vi "N-216 Stage Engine.vi"(0 "Unique Notifier Name":string, 11 "COM Port":string[](array[string])) -> ()   [LabVIEW 2016]
uses:
  Stages Controls/Stage Focus Control.ctl
  Stages Controls/Stage Status.ctl
  Stages Controls/Stage Actions.ctl
  Stages Controls/Stage Notifier Element.ctl
  PI GCS2 DLL/PI_GCS2_DLL_x64.dll
panel:
  in  "Reference":bool
  in  "Velocity (µm/s)":dbl=0.1 format="%#_13g"
  out "Number Connected":i32
  out "E-712 Found":bool
  in  "ReInitialize":bool
  in  "Abort":bool
  out "Status":T1
  in  "QUIT":bool
  in  "Focus Control":T2
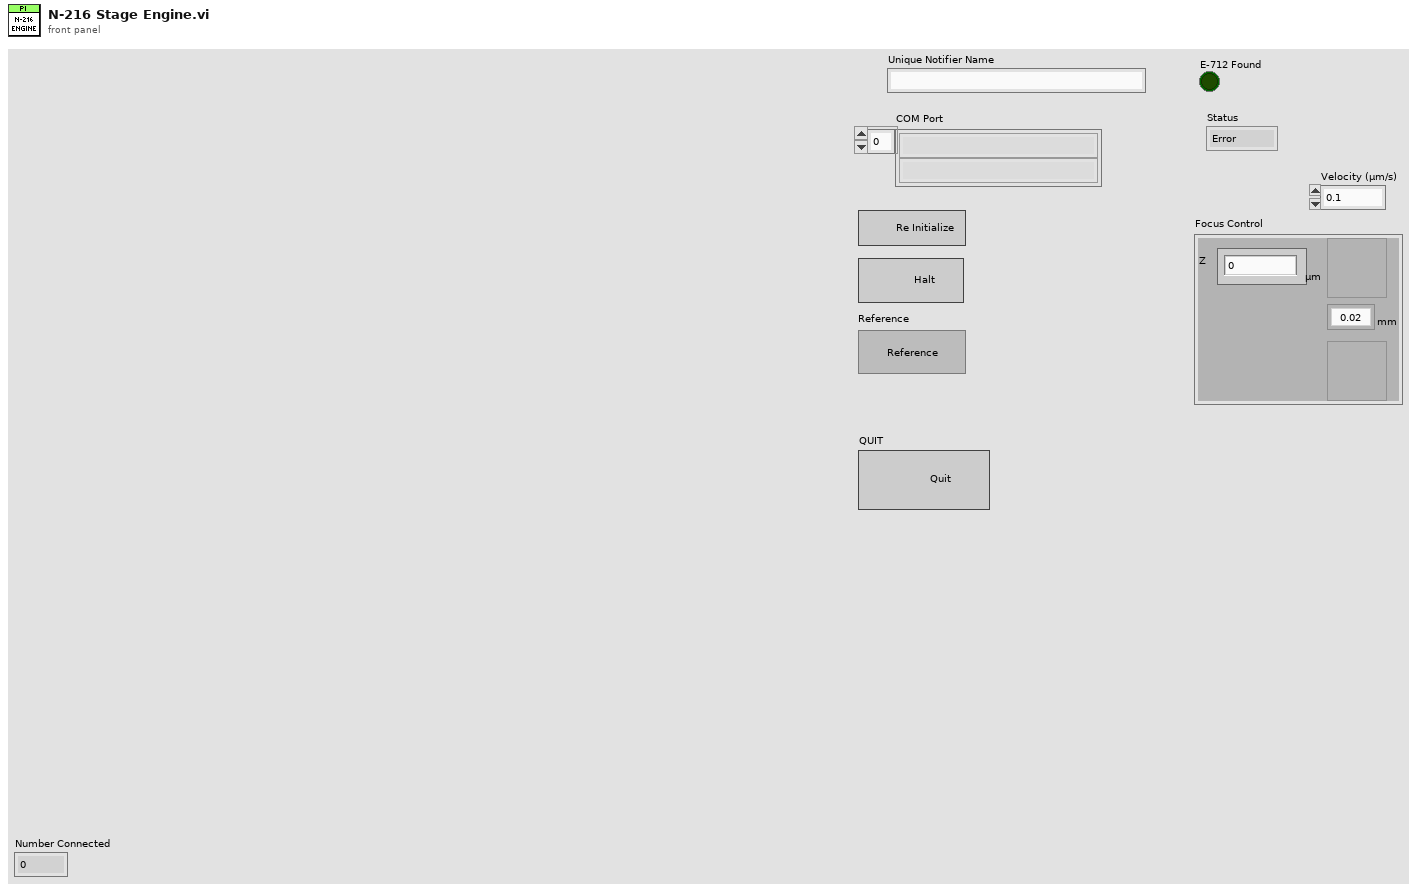
[diagram p1: front panel]
types:
  T1 = typedef "Stage Status.ctl" = enum16{"Error", "Abort", "Busy", "On Target"}
  T2 = typedef "Stage Focus Control.ctl" = cluster{"Focus Step (um)":enum16{"0.02", "0.05", "0.1", "0.5", "1", "2", "5", "10", "20"}, "Focus Up":bool, "Focus Down":bool, "Z ":dbl}
  T3 = typedef "Stage Notifier Element.ctl" = cluster{"Action":T4, "Axis":bool[], "Setpoint":dbl[], "Velocity":dbl, "Cmd Recvd?":bool, "Position":dbl[], "Status":T1, "Misc":variant}
  T4 = typedef "Stage Actions.ctl" = enum16{"Get Position", "MVR", "MOVE", "HALT", "ONTARGET", "ERROR", "REFERENCE", "INIT", "VELOCITY", "STATUS", "EXIT", "HOME", "ZEROPOS", "NANOPOS", "ANALOG", "QUIT"}
  T5 = enum32{"Invalid", "Standard", "Closed", "Hidden", "Minimized", "Maximized"}
  T6 = cluster{"Focus Step (um)":bool, "Focus Up":bool, "Focus Down":bool, "Z ":bool}
  T7 = enum16{"0.02", "0.05", "0.1", "0.5", "1", "2", "5", "10", "20"}
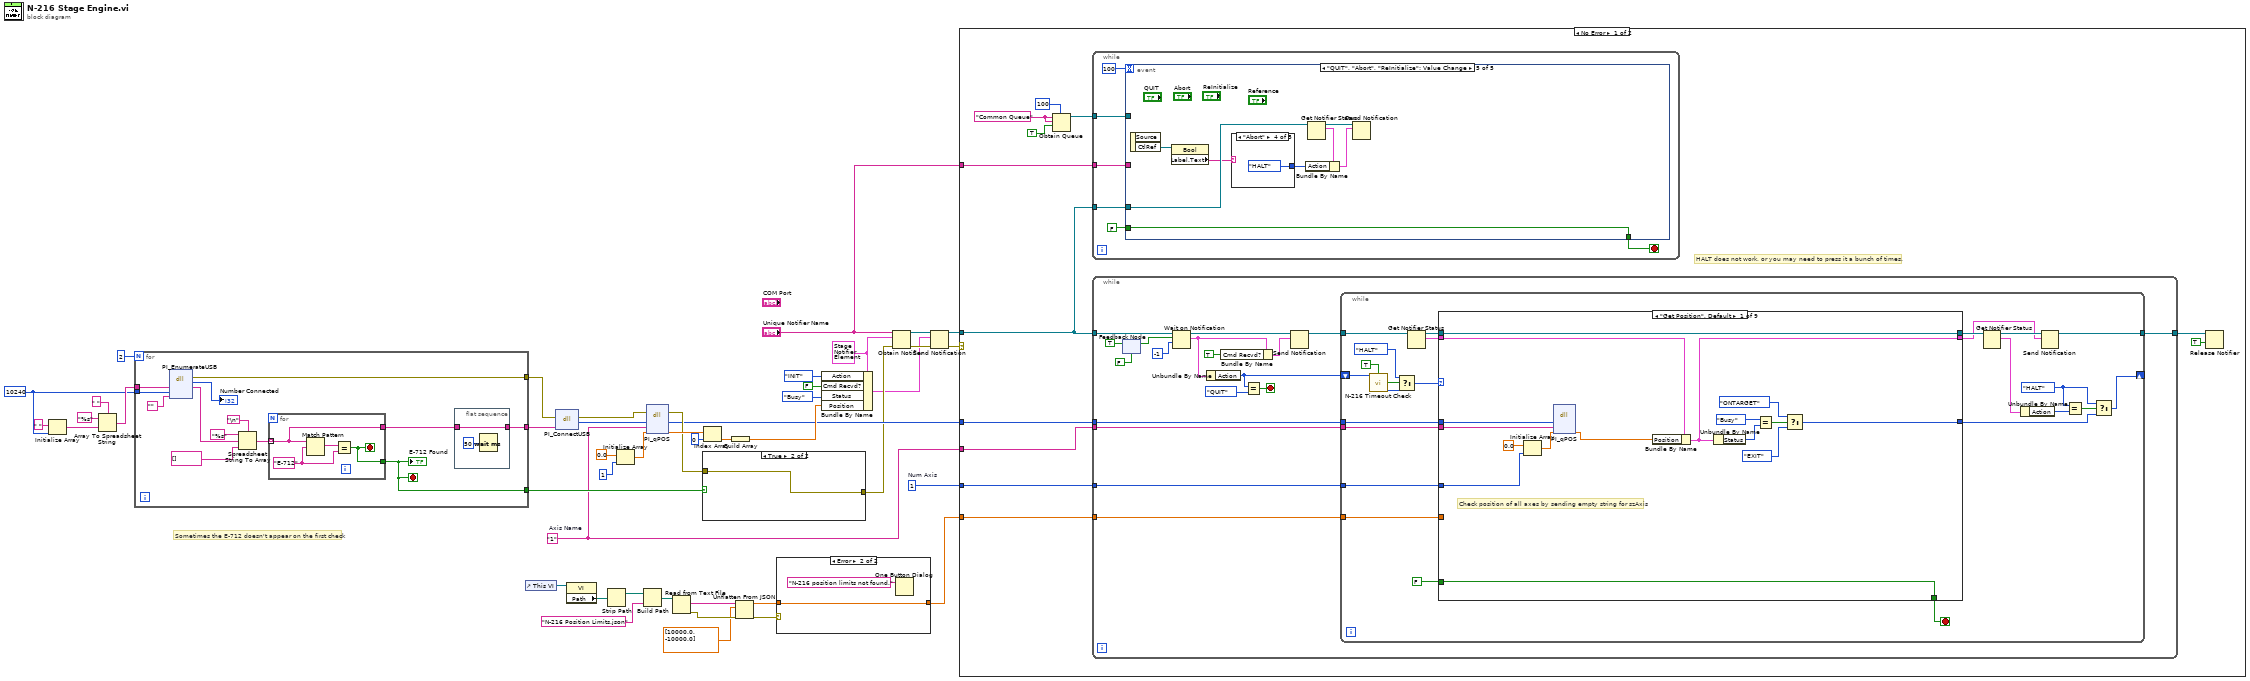
[diagram p0: block diagram]
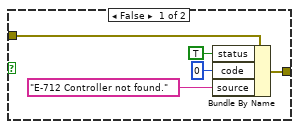
[diagram p3: hidden frame]
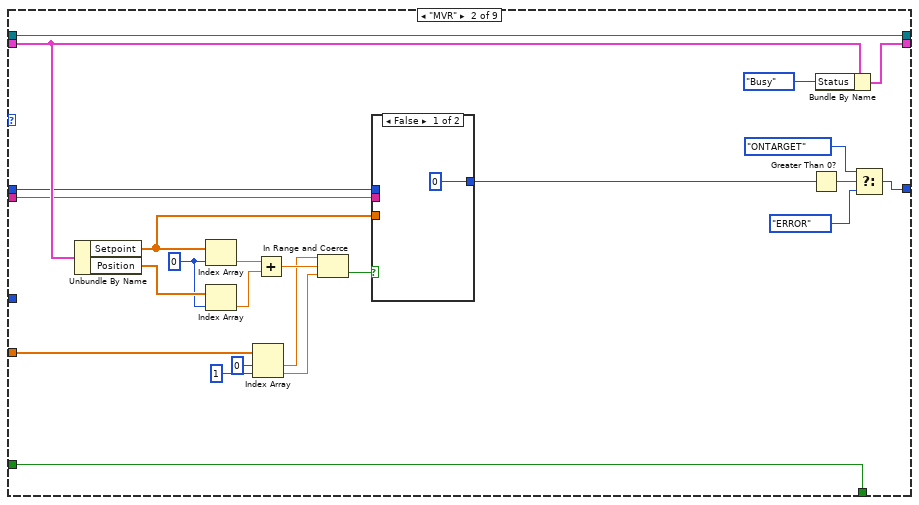
[diagram p4: hidden frame]
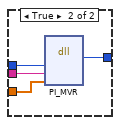
[diagram p5: hidden frame]
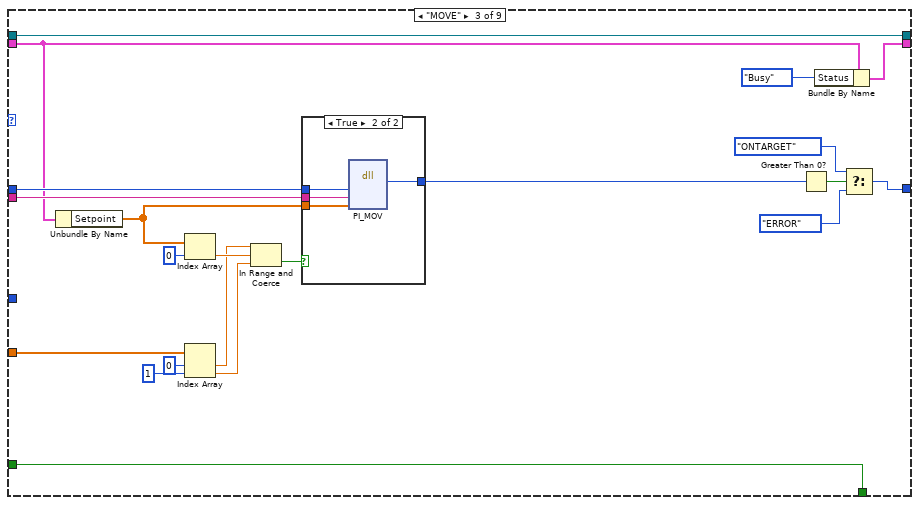
[diagram p6: hidden frame]
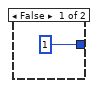
[diagram p7: hidden frame]
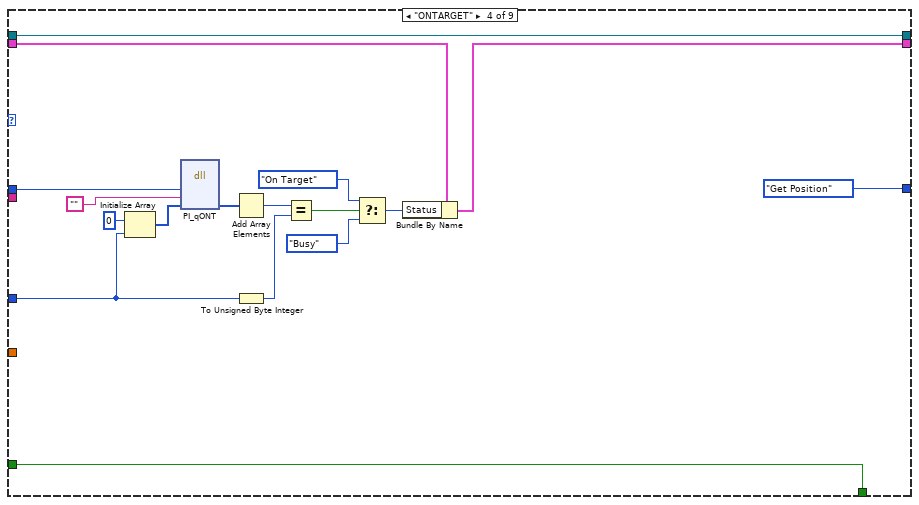
[diagram p8: hidden frame]
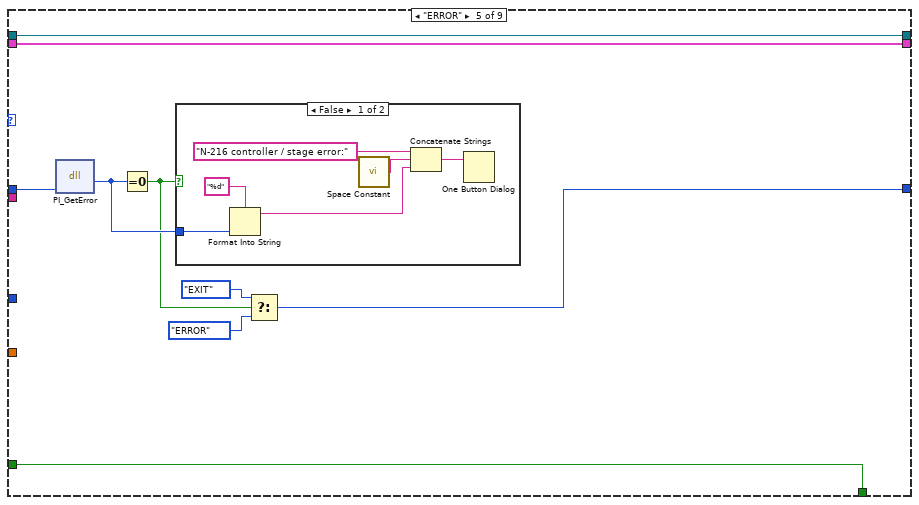
[diagram p9: hidden frame]
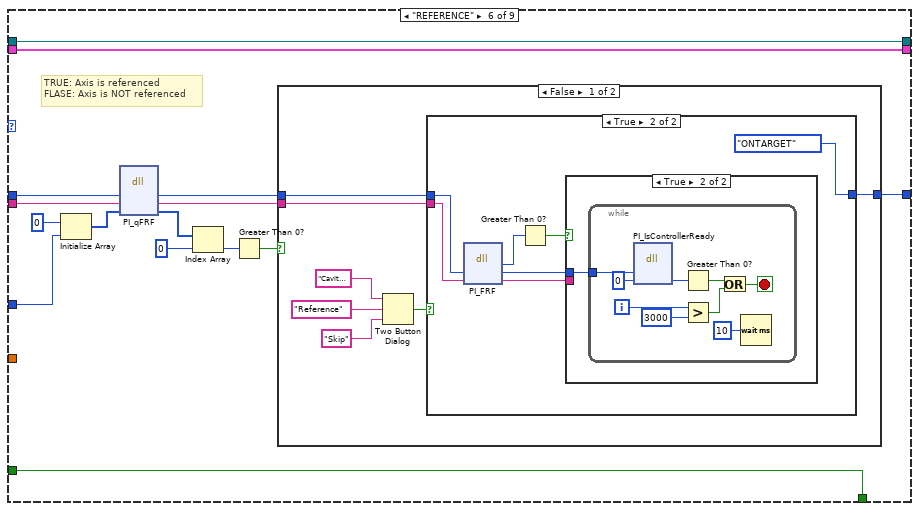
[diagram p11: hidden frame]
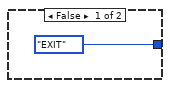
[diagram p12: hidden frame]
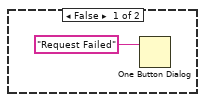
[diagram p13: hidden frame]
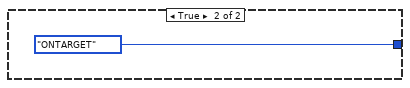
[diagram p14: hidden frame]
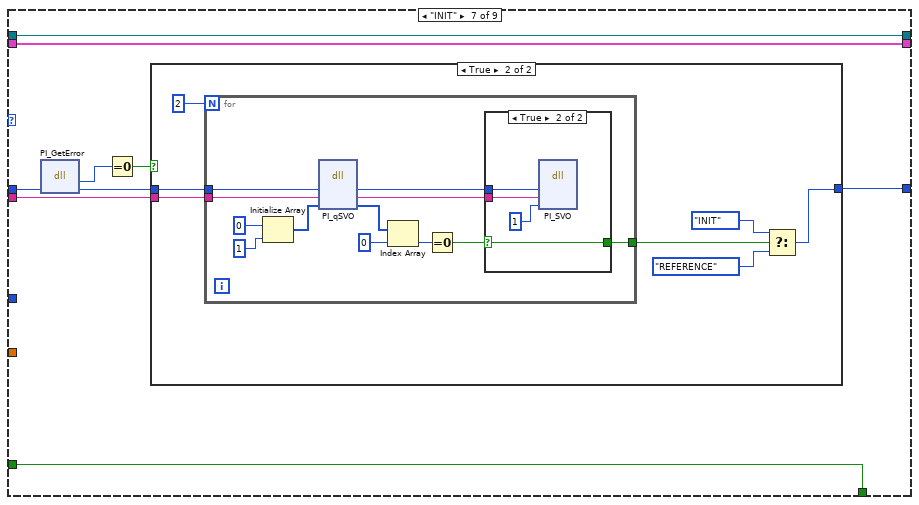
[diagram p15: hidden frame]
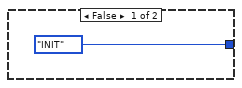
[diagram p16: hidden frame]
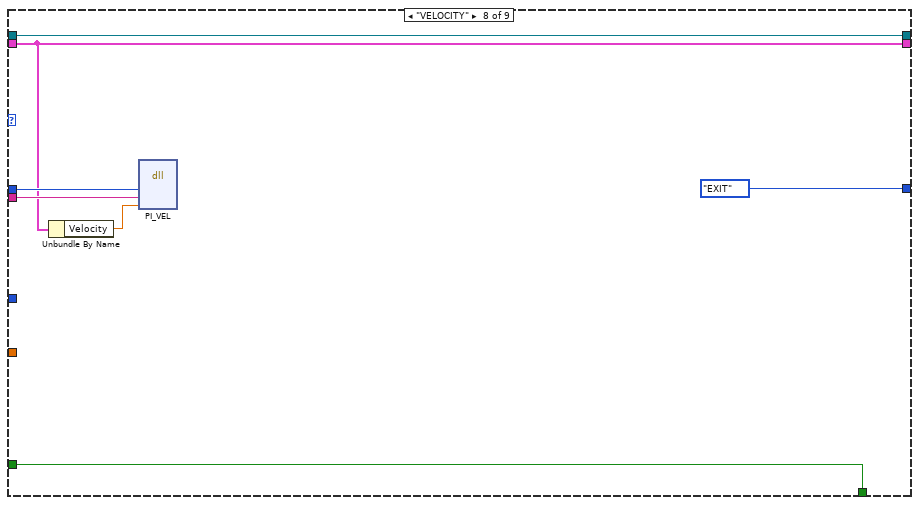
[diagram p18: hidden frame]
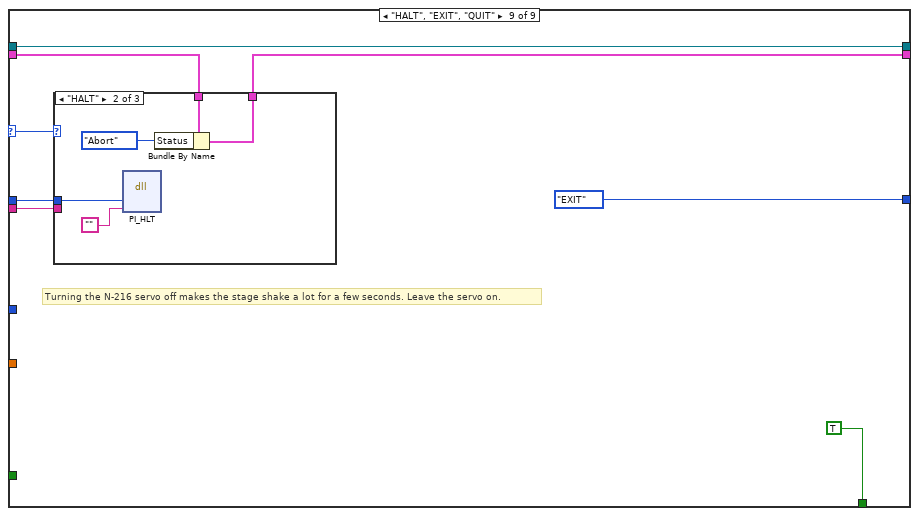
[diagram p19: hidden frame]
diagram:
  w13 = 1  # Num Axis
  w12 = "1"  # Axis Name
  w26 = T3 {"Action"=enum."Get Position", "Axis"=[], "Setpoint"=[], "Velocity"=0.5, "Cmd Recvd?"=FALSE, "Position"=[], "Status"=enum."Abort", "Misc"=variant} ("Stage Status")
  w40 = 10240 ("dimension size")
  # "Sometimes the E-712 doesn't appear on the first check"
  n1 = Initialize Array(" ", w40) -> (w44:string[])
  n2 = Array To Spreadsheet String(delimiter (Tab)=" ", array=w44, 3:"%s" ("format string")) -> (spreadsheet string=w41:string)
  n3 = for {
    N: 2 -> [_]
    tunnel: w41 -> [w53]
    tunnel: w40 -> [w52]
    tunnel: [w48] -> w38
    tunnel: [w47] -> w22
    tunnel: [w46] -> w32
    stop <- w47 stop-if-true
    n4 = dll-call lib="C:/Users/George Sirinakis/Documents/Microscope-Control/Device Library/Stages/PI/PI GCS2 DLL/PI_GCS2_DLL_x64.dll" fn="PI_EnumerateUSB"("szBuffer"=w53, "iBufferSize"=w52, "szFilter"="") -> (error out=w46:errorcluster, "return type"=→"Number Connected":i32, "szBuffer"=w50:string)  [unwired: 5 in, 1 out]
    n5 = Spreadsheet String To Array(delimiter (Tab)="\n", format string="%s", spreadsheet string=w50, array type (2D Dbl)=string[] []) -> (array=w55:string[])
    n6 = for {
      tunnel: w55 -> [w62] mode=indexing
      tunnel: [w62] -> w49
      tunnel: [w61] -> w47
      stop <- w61 stop-if-true
      w63 = "E-712"
      n7 = Match Pattern(string=w62, regular expression=w63) -> (match substring=w64:string)  [unwired: 1 in, 3 out]
      n8 = Equal?(x=w64, y=w63) -> (x = y?=w61:bool)
    }
    "E-712 Found" <- w47
    n9 = flat-sequence {
      tunnel: w49 -> [w60]
      tunnel: [w60] -> w48
      frame #0 {
        n10 = Wait (ms)(milliseconds to wait=u32 50) -> ()  [unwired: 1 out]
      }
    }
  }
  n11 = control-ref of="This VI"() -> (w11:refnum<vi>)
  n12 = dll-call lib="C:/Users/George Sirinakis/Documents/Microscope-Control/Device Library/Stages/PI/PI GCS2 DLL/PI_GCS2_DLL_x64.dll" fn="PI_ConnectUSB"(error in=w32, "szDescription"=w38) -> (error out=w33:errorcluster, "Device ID"=w34:i32)  [unwired: 3 in, 1 out]
  n13 = property class="VI"(reference=w11) -> ("Path"=w10:path)  [unwired: 1 in, 2 out]
  n14 = Strip Path(path=w10) -> (stripped path=w9:path)  [unwired: 1 out]
  n15 = Initialize Array(0.0 ("element"), 1 ("dimension size")) -> (w35:dbl[])
  n16 = Build Path(base path=w9, name or relative path="N-216 Position Limits.json") -> (appended path=w7:path)
  n17 = dll-call lib="C:/Users/George Sirinakis/Documents/Microscope-Control/Device Library/Stages/PI/PI GCS2 DLL/PI_GCS2_DLL_x64.dll" fn="PI_qPOS"(error in=w33, "Device ID"=w34, "szAxes"=w12, "pdValueArray"=w35) -> (error out=w21:errorcluster, "Device ID"=w20:i32, "pdValueArray"=w31:dbl[])  [unwired: 4 in, 1 out]
  n18 = Read from Text File(file (use dialog)=w7) -> (text=w6:string, error out=w5:errorcluster)  [unwired: 3 in, 2 out]
  n19 = case shown="True" w22 {
    tunnel: w21 -> [w69 w70]
    tunnel: [w67 w70] -> w19
    frame False {
      n20 = Bundle By Name(cluster=w69, "status"=TRUE, "code"=0, "source"="E-712 Controller not found.") -> (w67:errorcluster)
    }
    frame True {
    }
  }
  n21 = Index Array(array=w31, index=0) -> (element=w24:dbl)
  n22 = Build Array(w24) -> (w23:dbl[])
  n23 = Unflatten From JSON(JSON string=w6, type and defaults=dbl[] [10000.0, -10000.0], error in (no error)=w5) -> (value=w2:dbl[], error out=w3:errorcluster)  [unwired: 4 in]
  n24 = case shown="Error" w3 {
    tunnel: w2 -> [w71 w73]
    tunnel: [w71 w73] -> w1
    frame No Error {
    }
    frame Error {
      n25 = One Button Dialog(message="N-216 position limits not found.") -> ()  [unwired: 1 in, 1 out]
    }
  }
  n26 = Bundle By Name(cluster=w26, "Action"=Stage_Actions."INIT", "Cmd Recvd?"=FALSE, "Status"=Stage_Status."Busy", "Position"=w23) -> (w14:T3)
  n27 = Obtain Notifier(name (unnamed)="Unique Notifier Name", notification data type=w26, error in (no error)=w19) -> (notifier out=w18:refnum<notifier>, error out=w17:errorcluster)  [unwired: 1 in, 1 out]
  n28 = Send Notification(notification=w14, notifier=w18, error in (no error)=w17) -> (notifier out=w16:refnum<notifier>, error out=w15:errorcluster)
  n29 = case shown="No Error" w15 {
    selector: w15 -> [_ w429]
    tunnel: w16 -> [w79 w431]
    tunnel: "Unique Notifier Name" -> [w80 _]
    tunnel: w20 -> [w78 w430]
    tunnel: w12 -> [w77 _]
    tunnel: w13 -> [w75 _]
    tunnel: w1 -> [w74 _]
    frame No Error {
      w84 = "Common Queue" ("Unique Notifier Name")
      # "HALT does not work, or you may need to press it a bunch of times."
      n30 = Obtain Queue(max queue size (-1, unlimited)=100, name (unnamed)=w84, element data type=w84, create if not found? (T)=TRUE) -> (queue out=w81:refnum<queue>)  [unwired: 1 in, 2 out]
      n31 = while {
        tunnel: w79 -> [w341]
        tunnel: w81 -> [w340]
        tunnel: w80 -> [w339]
        stop <- w342 stop-if-true
        n32 = event shown="[4] \"QUIT\", \"Abort\", \"ReInitialize\": Value Change" {
          selector: _ -> [_ _ _ _ _]
          dyn-events: _ -> [_ _ _ _ _]
          timeout: 100 -> [_ _ _ _ _]
          tunnel: [w347 w360 w365 w414 w419] -> w342
          tunnel: w341 -> [w356 _ w370 w413 w422]
          tunnel: w340 -> [w349 _ _ _ _]
          tunnel: w339 -> [w344 _ _ _ _]
          tunnel: FALSE -> [_ w360 w365 w414 w419]
          event Timeout {
            n33 = event-data() -> ()  [unwired: 1 in, 1 out]
            n34 = call "Common Device Queue Get Command.vi"("Common Queue"=w349, "Notifier Name"=w344) -> ("Command"=w350:string)  [unwired: 12 in, 1 out]
            n35 = control-ref of="This VI"() -> (w351:refnum<vi>)
            n36 = call "Common Device Queue Execute Command.vi"("Common Command"=w350, "VI Refnum"=w351) -> ("Quit?"=w346:bool)  [unwired: 12 in, 1 out]
            n37 = Get Notifier Status(notifier=w356) -> (notifier out=w345:refnum<notifier>, current notification=w355:T3, error out=w353:errorcluster)  [unwired: 1 in, 2 out]
            n38 = Unbundle By Name(w355) -> ("Position"=w354:dbl[], "Status"=→"Status":T1)
            n39 = Unbundle By Name(w353) -> ("status"=w348:bool)
            n40 = Index Array(array=w354) -> (element=w357:dbl)  [unwired: 1 in]
            n41 = property on="Z" class="DigNum (strict)"("Value"=w357) -> ()  [unwired: 2 in, 2 out]
            n42 = Or(x=w346, y=w348) -> (x .or. y?=w347:bool)
            n43 = case shown="False" w346 {
              tunnel: w345 -> [_ w359]
              frame False {
              }
              frame True {
                n44 = Send Notification(notification=T3 {"Action"=enum."QUIT", "Axis"=[], "Setpoint"=[], "Velocity"=0.5, "Cmd Recvd?"=FALSE, "Position"=[], "Status"=enum."Error", "Misc"=variant} ("Stage Status"), notifier=w359) -> ()  [unwired: 1 in, 2 out]
              }
            }
          }
          event Application Instance Close? {
            n45 = event-data() -> ()  [unwired: 1 in, 5 out]
            n46 = control-ref of="This VI"() -> (w362:refnum<vi>)
            n47 = invoke class="VI" method="FP.Open"(reference=w362, "Activate"=TRUE ("Activate?"), "State"=T5."Standard") -> ()  [unwired: 2 in, 5 out]
            n48 = event-data("Discard?"=TRUE) -> ()  [unwired: 1 in, 1 out]
          }
          event Value Change {
            n49 = event-data() -> ("CtlRef"=w380:refnum<vi>, "OldVal"=w381:T2, "NewVal"=w374:T2)  [unwired: 1 in]
            n50 = Not Equal?(x=w381, y=w374) -> (x != y?=w379:T6)
            n51 = property class="Clust"(reference=w380) -> ("Controls[]"=w377:refnum<vi>[])  [unwired: 1 in, 2 out]
            n52 = Cluster To Array(cluster=w379) -> (array=w378:bool[])
            n53 = for {
              tunnel: w378 -> [w407] mode=indexing
              tunnel: [w406] -> w376
              tunnel: w377 -> [w406] mode=indexing
              stop <- w407 stop-if-true
            }
            n54 = property class="Ctl"(reference=w376) -> ("ClassName"=w375:string, "Label.Text"=w373:string)  [unwired: 1 in, 2 out]
            n55 = case shown="\"Boolean\"" w375 {
              tunnel: w374 -> [w389 w401 _]
              tunnel: w373 -> [w390 _ _]
              tunnel: [w384 w399 dbl[] []] -> w372
              tunnel: [w383 w398 w404] -> w371
              tunnel: [Stage_Actions."MVR" ("Action") Stage_Actions."MOVE" ("Action") Stage_Actions."Get Position" ("Action")] -> w369
              frame "Boolean" {
                n56 = Unbundle By Name(w389) -> ("Focus Step (um)"=w387:T7)
                n57 = Format Into String(w387) -> (resulting string=w388:string)  [unwired: 3 in, 1 out]
                n58 = Fract/Exp String To Number(string=w388) -> (number=w386:dbl)  [unwired: 3 in, 1 out]
                n59 = case shown="Default" w390 {
                  tunnel: w386 -> [w393 w394 w395]
                  tunnel: [w392 w394 w395] -> w385
                  frame "Focus Down" {
                    n60 = Negate(x=w393) -> (-x=w392:dbl)
                  }
                  frame "Focus Up" {
                  }
                  frame Default {
                  }
                }
                n61 = Build Array(w385) -> (w384:dbl[])
                n62 = Build Array(TRUE) -> (w383:bool[])
              }
              frame "Digital" {
                n63 = Unbundle By Name(w401) -> ("Z"=w400:dbl)
                n64 = Build Array(w400) -> (w399:dbl[])
                n65 = Build Array(TRUE) -> (w398:bool[])
              }
              frame Default {
                n66 = Build Array(FALSE) -> (w404:bool[])
              }
            }
            n67 = Get Notifier Status(notifier=w370) -> (notifier out=w368:refnum<notifier>, current notification=w367:T3)  [unwired: 1 in, 3 out]
            n68 = Bundle By Name(cluster=w367, "Action"=w369, "Setpoint"=w372, "Axis"=w371) -> (w366:T3)
            n69 = Send Notification(notification=w366, notifier=w368) -> ()  [unwired: 1 in, 2 out]
          }
          event "Velocity (µm/s)": Value Change {
            n70 = event-data() -> ("NewVal"=w410:dbl)  [unwired: 1 in]
            n71 = Get Notifier Status(notifier=w413) -> (notifier out=w409:refnum<notifier>, current notification=w412:T3)  [unwired: 1 in, 3 out]
            n72 = Bundle By Name(cluster=w412, "Action"=Stage_Actions."VELOCITY", "Velocity"=w410) -> (w408:T3)
            n73 = Send Notification(notification=w408, notifier=w409) -> ()  [unwired: 1 in, 2 out]
          }
          event "QUIT", "Abort", "ReInitialize": Value Change {
            n74 = event-data() -> ("CtlRef"=w421:refnum<vi>)  [unwired: 1 in, 1 out]
            n75 = property class="Bool"(reference=w421) -> ("Label.Text"=w420:string)  [unwired: 1 in, 2 out]
            n76 = case shown="\"Abort\"" w420 {
              tunnel: [Stage_Actions."EXIT" ("Action") Stage_Actions."QUIT" ("Action") Stage_Actions."INIT" ("Action") Stage_Actions."HALT" ("Action") Stage_Actions."REFERENCE" ("Action")] -> w418
              frame "Default", Default {
              }
              frame "QUIT" {
              }
              frame "ReInitialize" {
              }
              frame "Abort" {
              }
              frame "Reference" {
              }
            }
            n77 = Get Notifier Status(notifier=w422) -> (notifier out=w416:refnum<notifier>, current notification=w415:T3)  [unwired: 1 in, 3 out]
            n78 = Bundle By Name(cluster=w415, "Action"=w418) -> (w417:T3)
            n79 = Send Notification(notification=w417, notifier=w416) -> ()  [unwired: 1 in, 2 out]
          }
        }
      }
      n80 = while {
        tunnel: w79 -> [w100]
        tunnel: w78 -> [w98]
        tunnel: w77 -> [w97]
        tunnel: [w91] -> w76
        tunnel: w75 -> [w87]
        tunnel: w74 -> [w86]
        stop <- w103 stop-if-true
        n81 = feedback #1(FALSE) -> (w88:bool)
        n82 = feedback-in #1(TRUE) -> ()
        n83 = Wait on Notification(notifier=w100, ignore previous (F)=w88, timeout in ms (-1)=-1) -> (notifier out=w96:refnum<notifier>, notification=w94:T3)  [unwired: 1 in, 2 out]
        n84 = Unbundle By Name(w94) -> ("Action"=w99:T4)
        n85 = Bundle By Name(cluster=w94, "Cmd Recvd?"=TRUE) -> (w92:T3)
        n86 = Equal?(x=w99, y=Stage_Actions."QUIT") -> (x = y?=w103:bool)
        n87 = Send Notification(notification=w92, notifier=w96) -> (notifier out=w95:refnum<notifier>)  [unwired: 1 in, 1 out]
        n88 = while {
          tunnel: w98 -> [w126]
          tunnel: w95 -> [w118]
          shift-right: [w120] -> _
          shift-left: w99 -> [w113]
          tunnel: w97 -> [w125]
          tunnel: [w124] -> w91
          tunnel: w87 -> [w115]
          tunnel: w86 -> [w108]
          stop <- w127 stop-if-true
          w122 = Stage_Actions."HALT" ("Action")
          n89 = call "N-216 Timeout Check.vi"("Action"=w113, "User Input?"=TRUE) -> ("Timeout?"=w112:bool, "Action (Dup)"=w111:T4)  [unwired: 12 in]
          n90 = Select(t=Stage_Actions."HALT" ("y"), s=w112, f=w111) -> (s? t:f=w110:T4)
          n91 = Get Notifier Status(notifier=w118) -> (notifier out=w117:refnum<notifier>, current notification=w116:T3)  [unwired: 1 in, 3 out]
          n92 = case shown="\"Get Position\", Default" w110 {
            selector: w110 -> [_ _ _ _ _ _ _ _ w317]
            tunnel: w117 -> [w132 w167 w194 w216 w225 w246 w275 w314 w320]
            tunnel: FALSE -> [w141 w168 w193 w215 w223 w244 w280 w313 _]
            tunnel: [w141 w168 w193 w215 w223 w244 w280 w313 TRUE] -> w127
            tunnel: [w134 w163 w186 Stage_Actions."Get Position" ("y") w217 w236 w276 Stage_Actions."EXIT" ("y") Stage_Actions."EXIT" ("y")] -> w119
            tunnel: w126 -> [w142 w153 w192 w214 w222 w243 w282 w312 w319]
            tunnel: w125 -> [w129 w152 w191 _ _ w239 w277 w311 w318]
            tunnel: [w132 w167 w194 w216 w225 w246 w275 w314 w320] -> w107
            tunnel: [w140 w161 w185 w200 w224 w245 w274 w310 w315] -> w104
            tunnel: w116 -> [w133 w160 w183 w204 w224 w245 w274 w310 w316]
            tunnel: w115 -> [w131 _ _ w208 _ w232 _ _ _]
            tunnel: w108 -> [_ w149 w176 _ _ _ _ _ _]
            frame "Get Position", Default {
              # "Check position of all axes by sending empty string for szAxis"
              n93 = Initialize Array(0.0 ("element"), w131) -> (w144:dbl[])
              n94 = dll-call lib="C:/Users/George Sirinakis/Documents/Microscope-Control/Device Library/Stages/PI/PI GCS2 DLL/PI_GCS2_DLL_x64.dll" fn="PI_qPOS"("Device ID"=w142, "szAxes"=w129, "pdValueArray"=w144) -> ("pdValueArray"=w130:dbl[])  [unwired: 6 in, 2 out]
              n95 = Bundle By Name(cluster=w133, "Position"=w130) -> (w140:T3)
              n96 = Unbundle By Name(w140) -> ("Status"=w139:T1)
              n97 = Equal?(x=Stage_Status."Busy", y=w139) -> (x = y?=w137:bool)
              n98 = Select(t=Stage_Actions."ONTARGET" ("y"), s=w137, f=Stage_Actions."EXIT" ("y")) -> (s? t:f=w134:T4)
            }
            frame "MVR" {
              w158 = 0 ("index")
              n99 = Unbundle By Name(w160) -> ("Setpoint"=w151:dbl[], "Position"=w159:dbl[])
              n100 = Index Array(array=w151, index=w158) -> (element=w157:dbl)
              n101 = Index Array(array=w159, index=w158) -> (element=w156:dbl)
              n102 = Index Array(array=w149, index #1=0 ("index"), index #2=1 ("index")) -> (element #1=w146:dbl, element #2=w145:dbl)
              n103 = Add(x=w157, y=w156) -> (x+y=w155:dbl)
              n104 = In Range and Coerce(upper limit=w146, x=w155, lower limit=w145) -> (In Range?=w154:bool)  [unwired: 1 out]
              n105 = case shown="False" w154 {
                tunnel: w153 -> [_ w173]
                tunnel: w152 -> [_ w172]
                tunnel: w151 -> [_ w171]
                tunnel: [u8 0 ("Success") w170] -> w150
                frame False {
                }
                frame True {
                  n106 = dll-call lib="C:/Users/George Sirinakis/Documents/Microscope-Control/Device Library/Stages/PI/PI GCS2 DLL/PI_GCS2_DLL_x64.dll" fn="PI_MVR"("Device ID"=w173, "szAxes"=w172, "pdValueArray"=w171) -> ("Success"=w170:u8)  [unwired: 6 in, 2 out]
                }
              }
              n107 = Greater Than 0?(x=w150) -> (x > 0?=w166:bool)
              n108 = Bundle By Name(cluster=w160, "Status"=Stage_Status."Busy") -> (w161:T3)
              n109 = Select(t=Stage_Actions."ONTARGET" ("Action"), s=w166, f=Stage_Actions."ERROR" ("Action")) -> (s? t:f=w163:T4)
            }
            frame "MOVE" {
              n110 = Unbundle By Name(w183) -> ("Setpoint"=w182:dbl[])
              n111 = Index Array(array=w182, index=0) -> (element=w180:dbl)
              n112 = Index Array(array=w176, index #1=0 ("index"), index #2=1 ("index")) -> (element #1=w175:dbl, element #2=w174:dbl)
              n113 = In Range and Coerce(upper limit=w175, x=w180, lower limit=w174) -> (In Range?=w179:bool)  [unwired: 1 out]
              n114 = case shown="True" w179 {
                tunnel: w192 -> [_ w199]
                tunnel: w191 -> [_ w198]
                tunnel: [u8 1 ("Success") w197] -> w190
                tunnel: w182 -> [_ w196]
                frame False {
                }
                frame True {
                  n115 = dll-call lib="C:/Users/George Sirinakis/Documents/Microscope-Control/Device Library/Stages/PI/PI GCS2 DLL/PI_GCS2_DLL_x64.dll" fn="PI_MOV"("Device ID"=w199, "szAxes"=w198, "pdValueArray"=w196) -> ("Success"=w197:u8)  [unwired: 6 in, 2 out]
                }
              }
              n116 = Greater Than 0?(x=w190) -> (x > 0?=w189:bool)
              n117 = Bundle By Name(cluster=w183, "Status"=Stage_Status."Busy") -> (w185:T3)
              n118 = Select(t=Stage_Actions."ONTARGET" ("Action"), s=w189, f=Stage_Actions."ERROR" ("Action")) -> (s? t:f=w186:T4)
            }
            frame "ONTARGET" {
              n119 = Initialize Array(u8 0 ("element"), w208) -> (w212:u8[])
              n120 = dll-call lib="C:/Users/George Sirinakis/Documents/Microscope-Control/Device Library/Stages/PI/PI GCS2 DLL/PI_GCS2_DLL_x64.dll" fn="PI_qONT"("Device ID"=w214, "szAxes"="", "pdValueArray"=w212) -> ("pdValueArray"=w210:u8[])  [unwired: 6 in, 2 out]
              n121 = Add Array Elements(numeric array=w210) -> (sum=w209:u8)
              n122 = To Unsigned Byte Integer(number=w208) -> (unsigned 8bit integer=w207:u8)
              n123 = Equal?(x=w209, y=w207) -> (x = y?=w206:bool)
              n124 = Select(t=Stage_Status."On Target" ("Status"), s=w206, f=Stage_Status."Busy" ("Status")) -> (s? t:f=w201:T1)
              n125 = Bundle By Name(cluster=w204, "Status"=w201) -> (w200:T3)
            }
            frame "ERROR" {
              n126 = dll-call lib="C:/Users/George Sirinakis/Documents/Microscope-Control/Device Library/Stages/PI/PI GCS2 DLL/PI_GCS2_DLL_x64.dll" fn="PI_GetError"("Device ID"=w222) -> ("Error Code"=w221:i32)  [unwired: 4 in, 2 out]
              n127 = Equal To 0?(x=w221) -> (x = 0?=w220:bool)
              n128 = case shown="False" w220 {
                tunnel: w221 -> [w229 _]
                frame False {
                  n129 = Format Into String(format string="%d", w229) -> (resulting string=w227:string)  [unwired: 2 in, 1 out]
                  n130 = call <vilib>:"Space Constant.vi"() -> ("String"=w230:string)
                  n131 = Concatenate Strings("N-216 controller / stage error:", w230, w227) -> (w226:string)
                  n132 = One Button Dialog(message=w226) -> ()  [unwired: 1 in, 1 out]
                }
                frame True {
                }
              }
              n133 = Select(t=Stage_Actions."EXIT", s=w220, f=Stage_Actions."ERROR" ("Action")) -> (s? t:f=w217:T4)
            }
            frame "REFERENCE" {
              # "TRUE: Axis is referenced\nFLASE: Axis is NOT referenced"
              n134 = Initialize Array(u8 0 ("element"), w232) -> (w241:u8[])
              n135 = dll-call lib="C:/Users/George Sirinakis/Documents/Microscope-Control/Device Library/Stages/PI/PI GCS2 DLL/PI_GCS2_DLL_x64.dll" fn="PI_qFRF"("Device ID"=w243, "szAxes"=w239, "pdValueArray"=w241) -> ("Device ID"=w234:i32, "szAxes"=w235:string, "pdValueArray"=w240:u8[])  [unwired: 4 in, 2 out]
              n136 = Index Array(array=w240, index=0) -> (element=w237:u8)
              n137 = Greater Than 0?(x=w237) -> (x > 0?=w233:bool)
              n138 = case shown="False" w233 {
                tunnel: [w247 Stage_Actions."ONTARGET" ("Action")] -> w236
                tunnel: w235 -> [w248 _]
                tunnel: w234 -> [w249 _]
                frame False {
                  n139 = Two Button Dialog(message="Cavity stage (N-216) is not referenced.", 1:"Skip" ("F button name (\"Cancel\")"), 2:"Reference" ("T button name (\"OK\")")) -> (T button?=w250:bool)
                  n140 = case shown="True" w250 {
                    tunnel: w249 -> [_ w255]
                    tunnel: w248 -> [_ w256]
                    tunnel: [Stage_Actions."EXIT" ("Action") Stage_Actions."ONTARGET" ("Action")] -> w247
                    frame False {
                    }
                    frame True {
                      n141 = dll-call lib="C:/Users/George Sirinakis/Documents/Microscope-Control/Device Library/Stages/PI/PI GCS2 DLL/PI_GCS2_DLL_x64.dll" fn="PI_FRF"("Device ID"=w255, "szAxes"=w256) -> ("Success"=w257:u8, "Device ID"=w259:i32, "szAxes"=w260:string)  [unwired: 3 in, 2 out]
                      n142 = Greater Than 0?(x=w257) -> (x > 0?=w258:bool)
                      n143 = case shown="True" w258 {
                        tunnel: w259 -> [_ w263]
                        tunnel: w260 -> [_ _]
                        frame False {
                          n144 = One Button Dialog(message="Request Failed") -> ()  [unwired: 1 in, 1 out]
                        }
                        frame True {
                          n145 = while {
                            tunnel: w263 -> [w272]
                            i -> [w270]
                            stop <- w265 stop-if-true
                            n146 = dll-call lib="C:/Users/George Sirinakis/Documents/Microscope-Control/Device Library/Stages/PI/PI GCS2 DLL/PI_GCS2_DLL_x64.dll" fn="PI_IsControllerReady"("Device ID"=w272, "piControllerReady"=0) -> ("piControllerReady"=w268:i32)  [unwired: 5 in, 2 out]
                            n147 = Greater Than 0?(x=w268) -> (x > 0?=w267:bool)
                            n148 = Greater?(x=w270, y=3000) -> (0:w266:bool)
                            n149 = Or(x=w267, y=w266) -> (x .or. y?=w265:bool)
                            n150 = Wait (ms)(milliseconds to wait=u32 10) -> ()  [unwired: 1 out]
                          }
                        }
                      }
                    }
                  }
                }
                frame True {
                }
              }
            }
            frame "INIT" {
              n151 = dll-call lib="C:/Users/George Sirinakis/Documents/Microscope-Control/Device Library/Stages/PI/PI GCS2 DLL/PI_GCS2_DLL_x64.dll" fn="PI_GetError"("Device ID"=w282) -> ("Error Code"=w281:i32, "Device ID"=w278:i32)  [unwired: 3 in, 2 out]
              n152 = Equal To 0?(x=w281) -> (x = 0?=w279:bool)
              n153 = case shown="True" w279 {
                tunnel: w278 -> [_ w290]
                tunnel: w277 -> [_ w289]
                tunnel: [Stage_Actions."INIT" ("Action") w286] -> w276
                frame False {
                }
                frame True {
                  n154 = for {
                    N: 2 -> [_]
                    tunnel: w290 -> [w299]
                    tunnel: w289 -> [w298]
                    tunnel: [w291] -> w287
                    n155 = Initialize Array(u8 0 ("element"), 1 ("dimension size")) -> (w302:u8[])
                    n156 = dll-call lib="C:/Users/George Sirinakis/Documents/Microscope-Control/Device Library/Stages/PI/PI GCS2 DLL/PI_GCS2_DLL_x64.dll" fn="PI_qSVO"("Device ID"=w299, "szAxes"=w298, "pdValueArray"=w302) -> ("Device ID"=w292:i32, "szAxes"=w293:string, "pdValueArray"=w297:u8[])  [unwired: 4 in, 2 out]
                    n157 = Index Array(array=w297, index=0) -> (element=w295:u8)
                    n158 = Equal To 0?(x=w295) -> (x = 0?=w294:bool)
                    n159 = case shown="True" w294 {
                      selector: w294 -> [w303 w304]
                      tunnel: w293 -> [_ w306]
                      tunnel: w292 -> [_ w307]
                      tunnel: [w303 w304] -> w291
                      frame False {
                      }
                      frame True {
                        n160 = dll-call lib="C:/Users/George Sirinakis/Documents/Microscope-Control/Device Library/Stages/PI/PI GCS2 DLL/PI_GCS2_DLL_x64.dll" fn="PI_SVO"("Device ID"=w307, "szAxes"=w306, "pdValueArray"=u8 1) -> ()  [unwired: 7 in, 2 out]
                      }
                    }
                  }
                  n161 = Select(t=Stage_Actions."INIT" ("Action"), s=w287, f=Stage_Actions."REFERENCE" ("Action")) -> (s? t:f=w286:T4)
                }
              }
            }
            frame "VELOCITY" {
              n162 = Unbundle By Name(w310) -> ("Velocity"=w309:dbl)
              n163 = dll-call lib="C:/Users/George Sirinakis/Documents/Microscope-Control/Device Library/Stages/PI/PI GCS2 DLL/PI_GCS2_DLL_x64.dll" fn="PI_VEL"("Device ID"=w312, "szAxes"=w311, "pdValueArray"=w309) -> ()  [unwired: 7 in, 2 out]
            }
            frame "HALT", "EXIT", "QUIT" {
              # "Turning the N-216 servo off makes the stage shake a lot for a few seconds. Leave the servo on."
              n164 = case shown="\"HALT\"" w317 {
                tunnel: w319 -> [_ w328 w332]
                tunnel: w318 -> [_ _ w331]
                tunnel: w316 -> [w323 w326 w329]
                tunnel: [w323 w324 w329] -> w315
                frame Default {
                }
                frame "HALT" {
                  n165 = dll-call lib="C:/Users/George Sirinakis/Documents/Microscope-Control/Device Library/Stages/PI/PI GCS2 DLL/PI_GCS2_DLL_x64.dll" fn="PI_HLT"("Device ID"=w328, "szAxes"="") -> ()  [unwired: 6 in, 2 out]
                  n166 = Bundle By Name(cluster=w326, "Status"=Stage_Status."Abort") -> (w324:T3)
                }
                frame "QUIT" {
                  n167 = disable-structure shown="Disabled" {
                    disable-tunnel: w332 -> [w335 w337]
                    disable-tunnel: w331 -> [w334 _]
                    disable-tunnel: [w333 w337] -> w330
                    frame Disabled {
                      n168 = dll-call lib="C:/Users/George Sirinakis/Documents/Microscope-Control/Device Library/Stages/PI/PI GCS2 DLL/PI_GCS2_DLL_x64.dll" fn="PI_SVO"("Device ID"=w335, "szAxes"=w334, "pdValueArray"=u8 0) -> ("Device ID"=w333:i32)  [unwired: 6 in, 2 out]
                    }
                    frame Enabled {
                    }
                  }
                  n169 = dll-call lib="C:/Users/George Sirinakis/Documents/Microscope-Control/Device Library/Stages/PI/PI GCS2 DLL/PI_GCS2_DLL_x64.dll" fn="PI_CloseConnection"("Device ID"=w330) -> ()  [unwired: 5 in, 2 out]
                }
              }
            }
          }
          n170 = Get Notifier Status(notifier=w107) -> (notifier out=w106:refnum<notifier>, current notification=w105:T3)  [unwired: 1 in, 3 out]
          n171 = Unbundle By Name(w105) -> ("Action"=w121:T4)
          n172 = Send Notification(notification=w104, notifier=w106) -> (notifier out=w124:refnum<notifier>)  [unwired: 1 in, 1 out]
          n173 = Equal?(x=w122, y=w121) -> (x = y?=w123:bool)
          n174 = Select(t=w122, s=w123, f=w119) -> (s? t:f=w120:T4)
        }
      }
      n175 = Release Notifier(notifier=w76, force destroy? (F)=TRUE) -> ()  [unwired: 1 in, 3 out]
    }
    frame Error {
      n176 = dll-call lib="C:/Users/George Sirinakis/Documents/Microscope-Control/Device Library/Stages/PI/PI GCS2 DLL/PI_GCS2_DLL_x64.dll" fn="PI_CloseConnection"(error in=w429, "Device ID"=w430) -> (error out=w428:errorcluster)  [unwired: 4 in, 1 out]
      n177 = Release Notifier(notifier=w431, force destroy? (F)=TRUE, error in (no error)=w428) -> (error out=w436:errorcluster)  [unwired: 2 out]
      n178 = Unbundle By Name(w436) -> ("source"=w433:string)
      n179 = Concatenate Strings("N-216 Initialization Error", "\r", w433) -> (w432:string)
      n180 = One Button Dialog(message=w432) -> ()  [unwired: 1 in, 1 out]
    }
  }
